vi "lvmcp_autoerr.vi"() -> ()   [LabVIEW 2026]
panel:
  out "error out":errorcluster
  in  "enabled":bool
  in  "reference":refnum<vi>
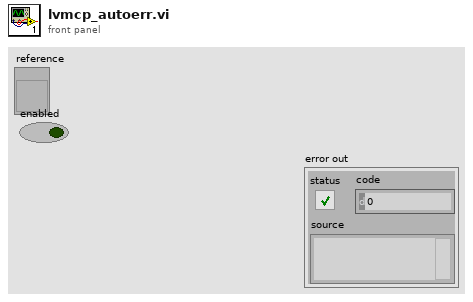
[diagram p1: front panel]
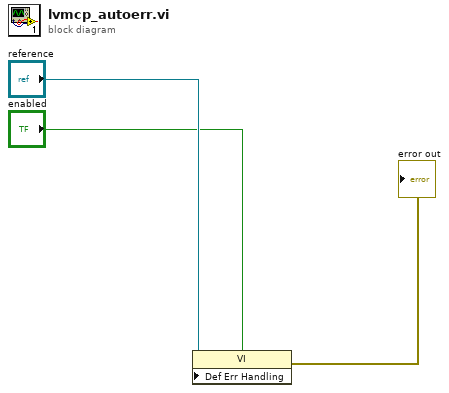
[diagram p0: block diagram]
diagram:
  n1 = property class="VI"(reference="reference", "Def Err Handling"="enabled") -> (error out=→"error out":errorcluster)  [unwired: 1 in, 1 out]
